vi "DAC Configure.vi"(8 "error in":errorcluster, 11 "DAC LN2 Temp in":refnum<class "DAC LN2 Temp.lvclass">) -> (0 "error out":errorcluster, 3 "DAC LN2 Temp out":refnum<class "DAC LN2 Temp.lvclass">)   [LabVIEW 2019, in "DAC.lvlib" / "DAC LN2 Temp.lvclass"]
uses:
  DAC LN2 Temp.lvclass
  DAC.lvclass
  <vilib>/DAQmx/create/channels.llb/DAQmx Create Channel (AI-Temperature-RTD).vi
  C:/Users/wg/Documents/LV_Projects/test-stand/App/DAC/DAC.lvclass
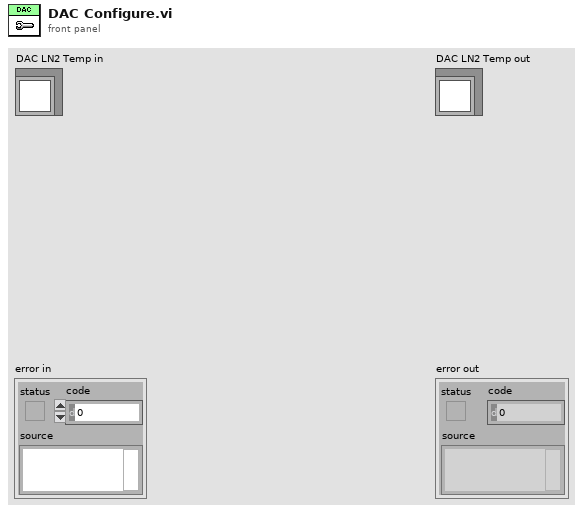
[diagram p1: front panel]
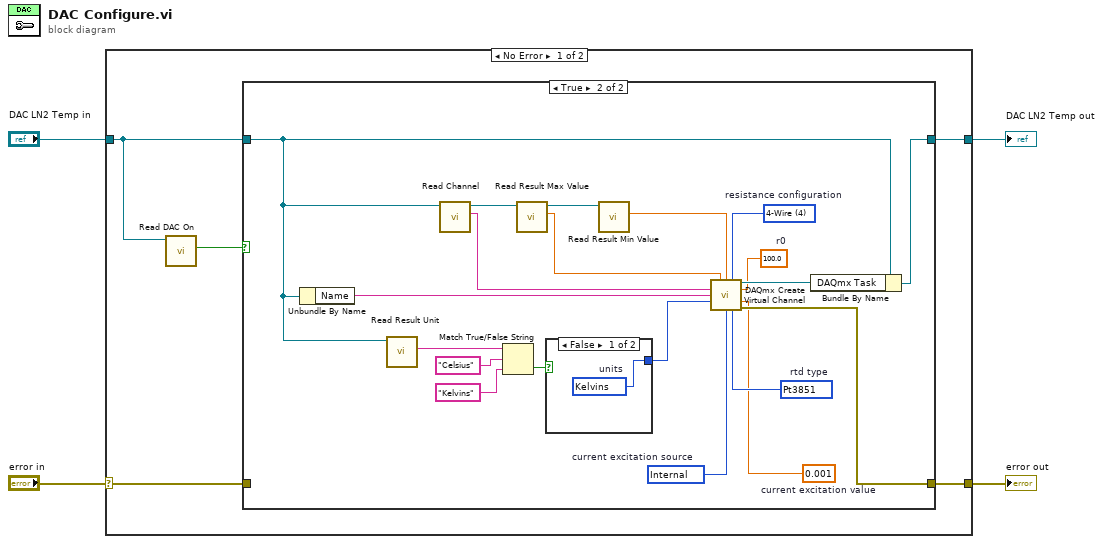
[diagram p0: block diagram]
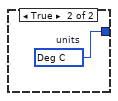
[diagram p3: hidden frame]
diagram:
  n1 = case shown="No Error" "error in" {
    selector: "error in" -> [w6 w35]
    tunnel: [w5 w35] -> w4
    tunnel: [w7 w34] -> w3
    tunnel: "DAC LN2 Temp in" -> [w9 w34]
    frame No Error {
      n2 = call "Read DAC On.vi"("DAC in"=w9) -> ("DAC On"=w8:bool)  [unwired: 8 in, 2 out]
      n3 = case shown="True" w8 {
        tunnel: w9 -> [w11 w17]
        tunnel: [w11 w31] -> w7
        tunnel: w6 -> [w10 _]
        tunnel: [w10 w28] -> w5
        frame False {
          # "Temperature measurement is off."
        }
        frame True {
          w23 = 0.001  # current excitation value
          w24 = 10071 items=["Pt3750"=12481, "Pt3851"=10071, "Pt3911"=12482, "Pt3916"=10069, "Pt3920"=10053, "Pt3928"=12483, "Custom"=10137]  # rtd type
          w25 = 10200 items=["Internal"=10200, "External"=10167, "None"=10230]  # current excitation source
          w26 = 100.0  # r0
          w27 = 4 items=["2-Wire"=2, "3-Wire"=3, "4-Wire"=4]  # resistance configuration
          # "Temperature measurement is on."
          n4 = Unbundle By Name(w17) -> ("Name"=w30:string)
          n5 = call "Read Result Unit.vi"("DAC in"=w17) -> ("Unit"=w19:string)  [unwired: 8 in, 2 out]
          n6 = call "Read Channel.vi"("DAC in"=w17) -> ("Channel"=w12:string, "DAC out"=w16:refnum<class "DAC LN2 Temp.lvclass">)  [unwired: 8 in, 1 out]
          n7 = Match True/False String(2:"Kelvins" ("false string"), 3:"Celsius" ("true string"), 4:w19) -> (0:w20:bool)  [unwired: 1 out]
          n8 = call "Read Result Max Value.vi"("DAC in"=w16) -> ("Max Value"=w13:dbl, "DAC out"=w15:refnum<class "DAC LN2 Temp.lvclass">)  [unwired: 8 in, 1 out]
          n9 = case shown="False" w20 {
            tunnel: [w32 w33] -> w18
            frame False {
              w32 = 10325 items=["Deg C"=10143, "Deg F"=10144, "Kelvins"=10325, "Deg R"=10145, "From Custom Scale"=10065]  # units
            }
            frame True {
              w33 = 10143 items=["Deg C"=10143, "Deg F"=10144, "Kelvins"=10325, "Deg R"=10145, "From Custom Scale"=10065]  # units
            }
          }
          n10 = call "Read Result Min Value.vi"("DAC in"=w15) -> ("Min Value"=w14:dbl)  [unwired: 8 in, 2 out]
          n11 = call-poly <vilib>:"DAQmx Create Virtual Channel.vi"("maximum value"=w13, "minimum value"=w14, "resistance configuration"=w27, "physical channels"=w12, "r0"=w26, "name to assign"=w30, "units"=w18, "current excitation value"=w23, "current excitation source"=w25, "rtd type"=w24) -> ("task out"=w29:refnum<k21>, "error out"=w28:errorcluster)  [unwired: 4 in]
          n12 = Bundle By Name(cluster=w17, "DAQmx Task"=w29) -> (w31:refnum<class "DAC LN2 Temp.lvclass">)
        }
      }
    }
    frame Error {
    }
  }
  "error out" <- w4
  "DAC LN2 Temp out" <- w3
